vi "FRC Check Project Names.vi"(8 "error in (no error)":errorcluster, 10 "project name":string, 11 "project folder":path) -> (0 "error out":errorcluster, 3 "proceed?":bool)   [LabVIEW 2027]
uses:
  <resource>/plugins/NewDialogFiles/ProjectWizards/FRC/FRC Strings.vi
panel:
  out "error out 2":errorcluster
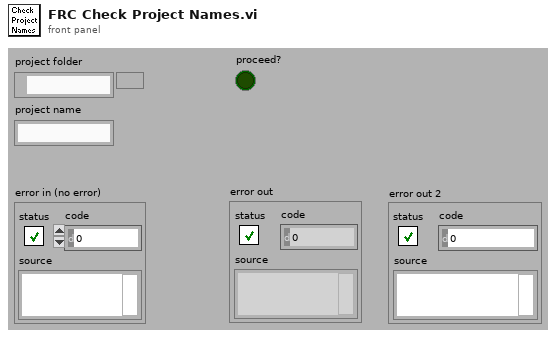
[diagram p1: front panel]
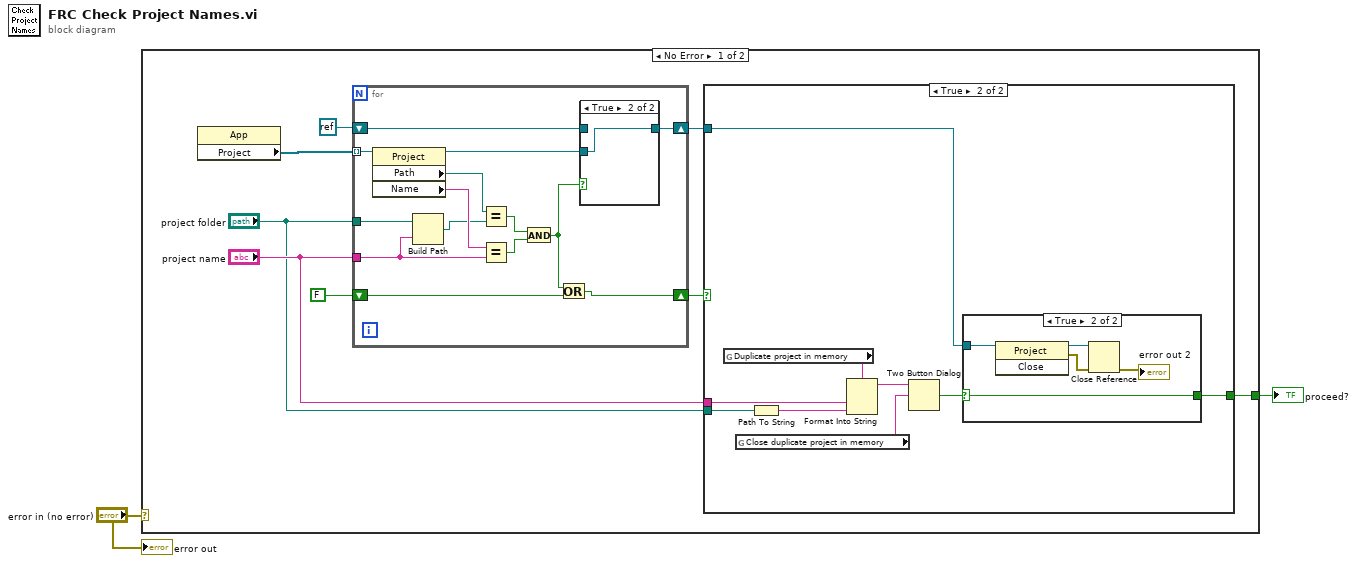
[diagram p0: block diagram]
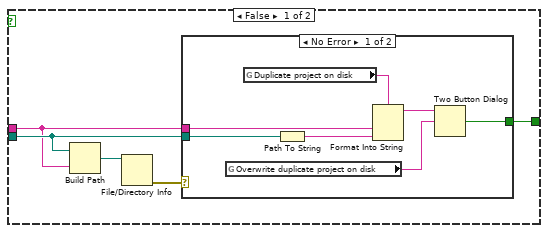
[diagram p2: hidden frame]
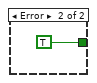
[diagram p3: hidden frame]
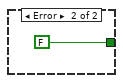
[diagram p6: hidden frame]
diagram:
  n1 = case shown="No Error" "error in (no error)" {
    tunnel: [w5 FALSE ("T button?")] -> w2
    frame No Error {
      n2 = property class="App"() -> ("Project"=w10:refnum<vi>[])  [unwired: 2 in, 2 out]
      n3 = for {
        tunnel: w10 -> [w52] mode=indexing
        shift-right: [w42] -> w8
        shift-left: FALSE -> [w50]
        tunnel: "project name" -> [w41]
        tunnel: "project folder" -> [w40]
        shift-right: [w45] -> w6
        shift-left: refnum<k0> refnum -> [w44]
        n4 = property class="Project"(reference=w52) -> (reference out=w46:refnum<vi>, "Path"=w51:path, "Name"=w49:string)  [unwired: 1 in, 1 out]
        n5 = Build Path(base path=w40, name or relative path=w41) -> (appended path=w39:path)
        n6 = Equal?(x=w51, y=w39) -> (x = y?=w47:bool)
        n7 = Equal?(x=w49, y=w41) -> (x = y?=w48:bool)
        n8 = And(x=w47, y=w48) -> (x .and. y?=w43:bool)
        n9 = Or(x=w43, y=w50) -> (x .or. y?=w42:bool)
        n10 = case shown="True" w43 {
          tunnel: [w53 w54] -> w45
          tunnel: w46 -> [_ w54]
          tunnel: w44 -> [w53 _]
          frame False {
          }
          frame True {
          }
        }
      }
      n11 = case shown="True" w8 {
        tunnel: "project name" -> [w13 w31]
        tunnel: "project folder" -> [w14 w30]
        tunnel: w6 -> [_ w25]
        tunnel: [w11 w24] -> w5
        frame False {
          n12 = Build Path(base path=w14, name or relative path=w13) -> (appended path=w15:path)
          n13 = File/Directory Info(path=w15) -> (error out=w12:errorcluster)  [unwired: 1 in, 6 out]
          n14 = case shown="No Error" w12 {
            tunnel: w14 -> [w18 _]
            tunnel: w13 -> [w17 _]
            tunnel: [w16 TRUE] -> w11
            frame No Error {
              n15 = global read "FRC Strings.vi" "Overwrite duplicate project on disk"() -> (w19:string)
              n16 = global read "FRC Strings.vi" "Duplicate project on disk"() -> (w20:string)
              n17 = Path To String(path=w18) -> (string=w22:string)
              n18 = Format Into String(format string=w20, w17, w22) -> (resulting string=w21:string)  [unwired: 2 in, 1 out]
              n19 = Two Button Dialog(message=w21, 2:w19) -> (T button?=w16:bool)  [unwired: 1 out]
            }
            frame Error {
            }
          }
        }
        frame True {
          n20 = global read "FRC Strings.vi" "Duplicate project in memory"() -> (w32:string)
          n21 = global read "FRC Strings.vi" "Close duplicate project in memory"() -> (w27:string)
          n22 = Path To String(path=w30) -> (string=w29:string)
          n23 = Format Into String(format string=w32, w31, w29) -> (resulting string=w28:string)  [unwired: 2 in, 1 out]
          n24 = Two Button Dialog(message=w28, 2:w27) -> (T button?=w26:bool)  [unwired: 1 out]
          n25 = case shown="True" w26 {
            selector: w26 -> [w33 w37]
            tunnel: w25 -> [_ w38]
            tunnel: [w33 w37] -> w24
            frame False {
            }
            frame True {
              n26 = invoke class="Project" method="Close"(reference=w38) -> (reference out=w36:refnum<vi>, error out=w35:errorcluster)  [unwired: 2 in, 1 out]
              n27 = Close Reference(reference=w36, error in (no error)=w35) -> (error out=→"error out 2":errorcluster)
            }
          }
        }
      }
    }
    frame Error {
    }
  }
  "proceed?" <- w2
  "error out" <- "error in (no error)"
